vi "csb ws parse frames.vi"(0 "state":u8[](array[numeric]), 1 "state_size":i32, 2 "in":u8[](array[numeric]), 3 "in_len":i32, 4 "opcodes":u8[](array[numeric]), 5 "lens":i32[](array[numeric]), 6 "max_frames":i32, 7 "error in (no error)":errorcluster, 8 "out":u8[](array[numeric]), 9 "out_cap":i32) -> (18 "out out":u8[](array[numeric]), 20 "state out":u8[](array[numeric]), 21 "n_frames":i32, 22 "function return":i32, 24 "opcodes out":u8[](array[numeric]), 25 "lens out":i32[](array[numeric]), 27 "error out":errorcluster)   [LabVIEW 2021, in "CANsub_Codec.lvlib"]
doc: "int32_t csb_ws_parse_frames(uint8_t *state, int32_t state_size,\n const uint8_t *in, int32_t in_len,\n uint8_t *opcodes, int32_t *lens, int32_t max_frames,\n uint8_t *out, int32_t out_cap, int32_t *n_frames);"
uses:
  CANsub_Codec.lvlib
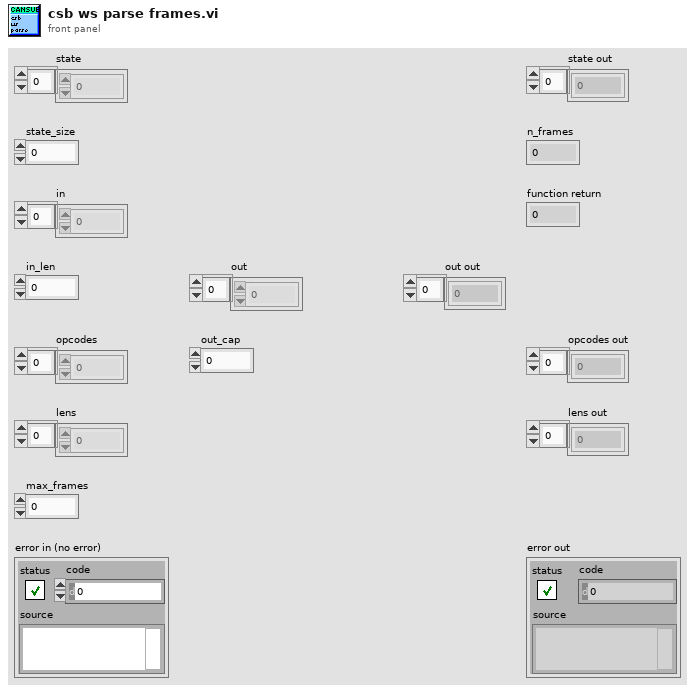
[diagram p1: front panel]
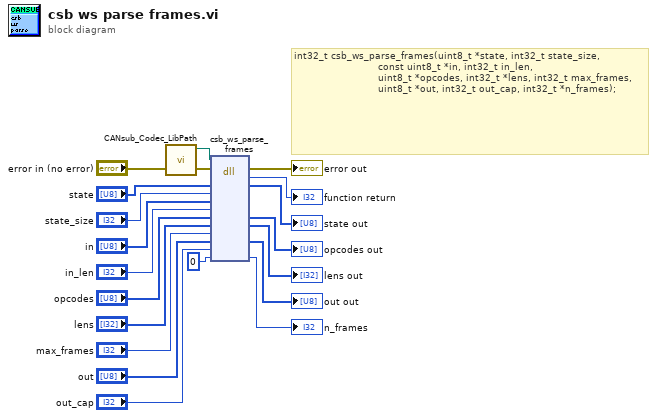
[diagram p0: block diagram]
diagram:
  # "int32_t csb_ws_parse_frames(uint8_t *state, int32_t state_size,\n                            const uint8_t *in, int32_t in_len,\n                            uint8_t *opcodes, int32_t *lens, int32_t max_frames,\n                            uint8_t *out, int32_t out_cap, int32_t *n_frames);"
  n1 = call "CANsub_Codec_LibPath.vi"() -> ("Path"=w1:path)  [unwired: 11 in]
  n2 = dll-call lib="libcansub_codec.*" fn="csb_ws_parse_frames"(path in=w1, error in="error in (no error)", "state"="state", "state_size"="state_size", "in"="in", "in_len"="in_len", "opcodes"="opcodes", "lens"="lens", "max_frames"="max_frames", "out"="out", "out_cap"="out_cap", "n_frames"=0) -> (error out=→"error out":errorcluster, "return type"=→"function return":i32, "state"=→"state out":u8[], "opcodes"=→"opcodes out":u8[], "lens"=→"lens out":i32[], "out"=→"out out":u8[], "n_frames"=→"n_frames":i32)  [unwired: 6 in, 1 out]
